vi "query IDN.vi"(8 "error in (no error)":errorcluster, 11 "FSV-40N in":refnum<class "FSV-40N.lvclass">) -> (0 "error out":errorcluster, 2 "Connected?":bool, 3 "FSV-40N out":refnum<class "FSV-40N.lvclass">)   [LabVIEW 2023, in "Spectrum Analyzer.lvlib" / "FSV-40N.lvclass"]
uses:
  FSV-40N.lvclass
  FSV-40N.lvclass/FSV-40N.ctl
  TYPE DEFINITION/TYPE Supported Spectrum Device Type.ctl
  Spectrum Analyzer.lvlib
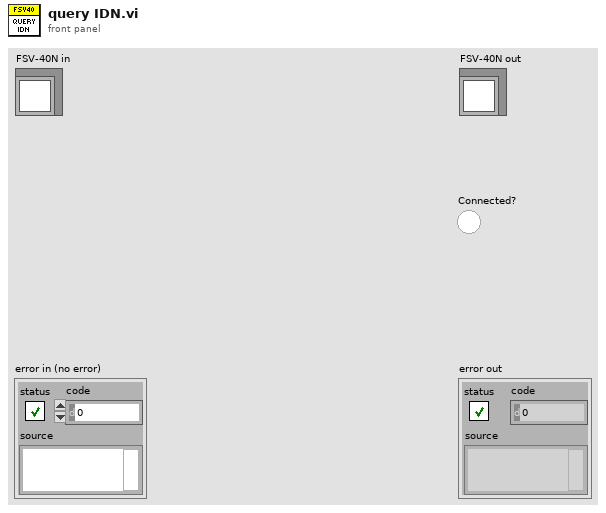
[diagram p1: front panel]
types:
  T1 = typedef "Spectrum Analyzer.lvlib/TYPE Supported Spectrum Device Type.ctl" = enum16{"None", "FSV-30", "FSV-40", "FSW", "9020A"}
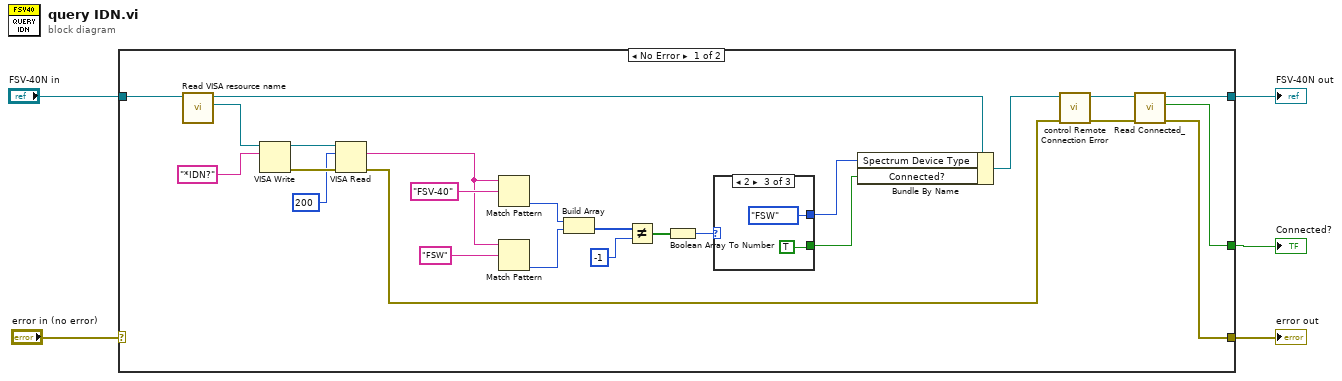
[diagram p0: block diagram]
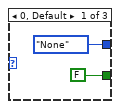
[diagram p2: hidden frame]
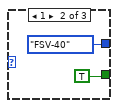
[diagram p3: hidden frame]
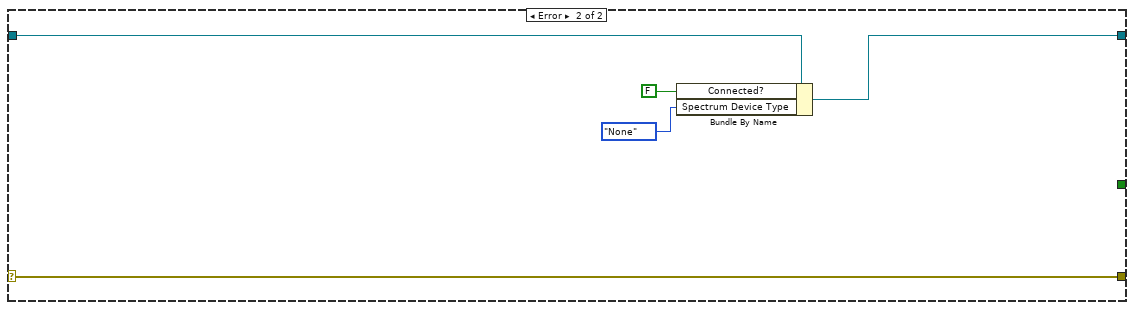
[diagram p4: hidden frame]
diagram:
  n1 = case shown="No Error" "error in (no error)" {
    selector: "error in (no error)" -> [_ w37]
    tunnel: "FSV-40N in" -> [w30 w41]
    tunnel: [w8 w38] -> w3
    tunnel: [w6 w37] -> w2
    tunnel: [w7 _] -> w1
    frame No Error {
      n2 = call "Read VISA resource name.vi"("FSV-40N in"=w30) -> ("VISA resource name"=w29:refnum<visa-resource-name>, "FSV-40N out"=w15:refnum<class "FSV-40N.lvclass">)  [unwired: 8 in, 1 out]
      n3 = VISA Write(VISA resource name=w29, write buffer="*IDN?") -> (VISA resource name out=w27:refnum<visa-resource-name>, error out=w26:errorcluster)  [unwired: 1 in, 1 out]
      n4 = VISA Read(VISA resource name=w27, byte count=u32 200, error in (no error)=w26) -> (read buffer=w23:string, error out=w11:errorcluster)  [unwired: 2 out]
      n5 = Match Pattern(string=w23, regular expression="FSV-40") -> (offset past match=w21:i32)  [unwired: 1 in, 3 out]
      n6 = Match Pattern(string=w23, regular expression="FSW") -> (offset past match=w20:i32)  [unwired: 1 in, 3 out]
      n7 = Build Array(w21, w20) -> (w19:i32[])
      n8 = Not Equal?(x=w19, y=-1) -> (x != y?=w17:bool[])
      n9 = Boolean Array To Number(Boolean array=w17) -> (number=w16:u32)
      n10 = case shown="2" w16 {
        tunnel: [FALSE TRUE TRUE] -> w13
        tunnel: [TYPE_Supported_Spectrum_Device_Type."None" ("Spectrum Device Type") TYPE_Supported_Spectrum_Device_Type."FSV-40" ("Spectrum Device Type") TYPE_Supported_Spectrum_Device_Type."FSW" ("Spectrum Device Type")] -> w14
        frame 0, Default {
        }
        frame 1 {
        }
        frame 2 {
        }
      }
      n11 = Bundle By Name(cluster=w15, "Spectrum Device Type"=w14, "Connected?"=w13) -> (w12:refnum<class "FSV-40N.lvclass">)
      n12 = call "control Remote Connection Error.vi"("error in (no error)"=w11, "FSV-40N in"=w12) -> ("error out"=w9:errorcluster, "FSV-40N out"=w10:refnum<class "FSV-40N.lvclass">)  [unwired: 8 in]
      n13 = call "Read Connected_.vi"("error in (no error)"=w9, "FSV-40N in"=w10) -> ("error out"=w6:errorcluster, "Connected?"=w7:bool, "FSV-40N out"=w8:refnum<class "FSV-40N.lvclass">)  [unwired: 7 in]
    }
    frame Error {
      n14 = Bundle By Name(cluster=w41, "Connected?"=FALSE, "Spectrum Device Type"=TYPE_Supported_Spectrum_Device_Type."None") -> (w38:refnum<class "FSV-40N.lvclass">)
    }
  }
  "error out" <- w2
  "FSV-40N out" <- w3
  "Connected?" <- w1
